vi "Open Pipe.vi"   [LabVIEW 2016, in "Linux RT IPC.Pipes.lvlib"]
doc: "This VI creates a new writer or reader endpoint for accessing the pipe and allowing data transfer."
uses:
  Linux RT IPC.Pipes.lvlib
  Classes/Unix Pipe Writer/Unix Pipe Writer.lvclass
  Classes/Unix Pipe Reader/Unix Pipe Reader.lvclass
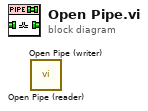
[diagram p0: block diagram]
diagram:
  n1 = call "Open Pipe (reader).vi"() -> ()  [unwired: 10 in, 2 out]
  n2 = call "Open Pipe (writer).vi"() -> ()  [unwired: 10 in, 2 out]
